vi "Virtual_Oscilloscope.vi"() -> ()   [LabVIEW 2020]
uses:
  <vilib>/Analysis/3filter.llb/Filter Passband Type.ctl
  <vilib>/Analysis/2dsp.llb/1D Convolution (DBL).vi
  <vilib>/measure/maspectr.llb/FFT Spectrum (Mag-Phase) for 1 Chan.vi
  <vilib>/Analysis/3filter.llb/Butterworth Filter (DBL).vi
  <vilib>/Analysis/3filter.llb/Chebyshev Filter (DBL).vi
  <vilib>/measure/NI_MABase.lvlib
  <vilib>/Analysis/NI_AALPro.lvlib
  <vilib>/Analysis/NI_AALBase.lvlib
  <vilib>/measure/NI_MAPro.lvlib
panel:
  in  "选项卡控件":enum32{"波形生成", "波形运算", "波形处理"}(tab)
  in  "占空比 3":dbl=50.0 caption="方波占空比(%)" format="%0.2f"
  in  "相位 3":dbl caption="相位" format="%.2p"
  in  "幅值 3":dbl=1.0 caption="幅值" format="%0.2p"
  in  "频率 3":dbl=10.0 caption="频率" format="%0.2p"
  out "CH1":waveform(dbl)(graph)
  in  "CH1波形":T1(ring)
  in  "CH1频率":i32(knob) scale=0.0..100.0
  in  "CH1幅值":i32(knob) scale=0.0..220.0
  in  "CH1相位":i32(knob) scale=0.0..180.0
  in  "CH1占空比":i32(knob) scale=0.0..100.0
  in  "采样数":dbl(slide) scale=1000.0..2000.0
  in  "采样频率":dbl(slide) scale=1000.0..2000.0
  in  "CH1-1":dbl(slide) scale=0.0..1.0
  in  "?":i32(knob) scale=1.0..7.0
  in  "Fs":dbl=1000.0 format="%.2p"
  in  "#s":dbl=1000.0 caption="采样数"
  in  "占空比 2":dbl=50.0 caption="方波占空比(%)" format="%0.2f"
  in  "相位 2":dbl caption="相位" format="%.2p"
  in  "幅值 2":dbl=1.0 caption="幅值" format="%0.2p"
  in  "频率 2":dbl=10.0 caption="频率" format="%0.2p"
  out "CH2":waveform(dbl)(graph)
  in  "CH2波形":T1(ring)
  in  "CH2-1":dbl(slide) scale=0.0..1.0
  in  "CH2幅值":i32(knob) scale=0.0..220.0
  in  "CH2相位":i32(knob) scale=0.0..180.0
  in  "CH2占空比":i32(knob) scale=0.0..100.0
  in  "CH2频率":i32(knob) scale=0.0..100.0
  in  "?":i32(knob) scale=1.0..7.0
  out "X-Y图":cluster{"Y":dbl[], "Y":dbl[]}(graph)
  in  "字符串":string
  in  "抵消":bool
  in  "叠加":bool
  in  "卷积":bool
  out "频率 5":dbl=10.0 caption="CH2频率" format="%0.2p"
  out "幅值 5":dbl=1.0 caption="CH2幅值" format="%0.2p"
  out "相位 5":dbl caption="CH2相位" format="%.2p"
  in  "处理后波形-1":dbl(slide) scale=0.0..1000.0
  in  "CH2-2":dbl(slide) scale=0.0..1.0
  out "处理后波形":dbl[](graph)
  out "CH2波形显示":waveform(dbl)(graph)
  out "CH1波形显示":waveform(dbl)(graph)
  in  "CH1-2":dbl(slide) scale=0.0..1.0
  out "频率 4":dbl=10.0 caption="CH1频率" format="%0.2p"
  out "幅值 4":dbl=1.0 caption="CH1幅值" format="%0.2p"
  out "相位 4":dbl caption="CH1相位" format="%.2p"
  out "滤波方式":enum16{"Butterworth", "Chebyshev"}(ring)
  out "滤波后FTT":cluster{"f0":dbl, "df":dbl, "magnitude":dbl[]}(graph)
  out "滤波后":dbl[](graph)
  in  "fh":dbl(slide) scale=1.0..10.0
  in  "FL":dbl(slide) scale=1.0..10.0
  in  "order":i32(knob) scale=0.0..10.0
  in  "fs":i32(knob) scale=0.0..100.0
  in  "滤波器类型":i32(knob) scale=1.0..4.0
  in  "滤波方式":i32(knob) scale=1.0..2.0
  in  "滤波后FTT":dbl(slide) scale=0.0..1.0
  out "滤波前FFT":cluster{"f0":dbl, "df":dbl, "magnitude":dbl[]}(graph)
  in  "滤波前FTT":dbl(slide) scale=0.0..1.0
  in  "滤波后":dbl(slide) scale=0.0..1000.0
  out "滤波前":dbl[](graph)
  in  "滤波前":dbl(slide) scale=0.0..1000.0
  in  "order":i32=2 caption="阶数"
  in  "filter type":T2 caption="滤波器类型"
  in  "low cutoff freq: fl":dbl=0.12500000000000006 caption="低截止频率:fl" format="%0.4f"
  in  "high cutoff freq: fh":dbl=0.45000000000000007 caption="高截止频率:fh" format="%0.2f"
  in  "sampling freq: fs":dbl=1.0 caption="采样频率:fs" format="%0.2f"
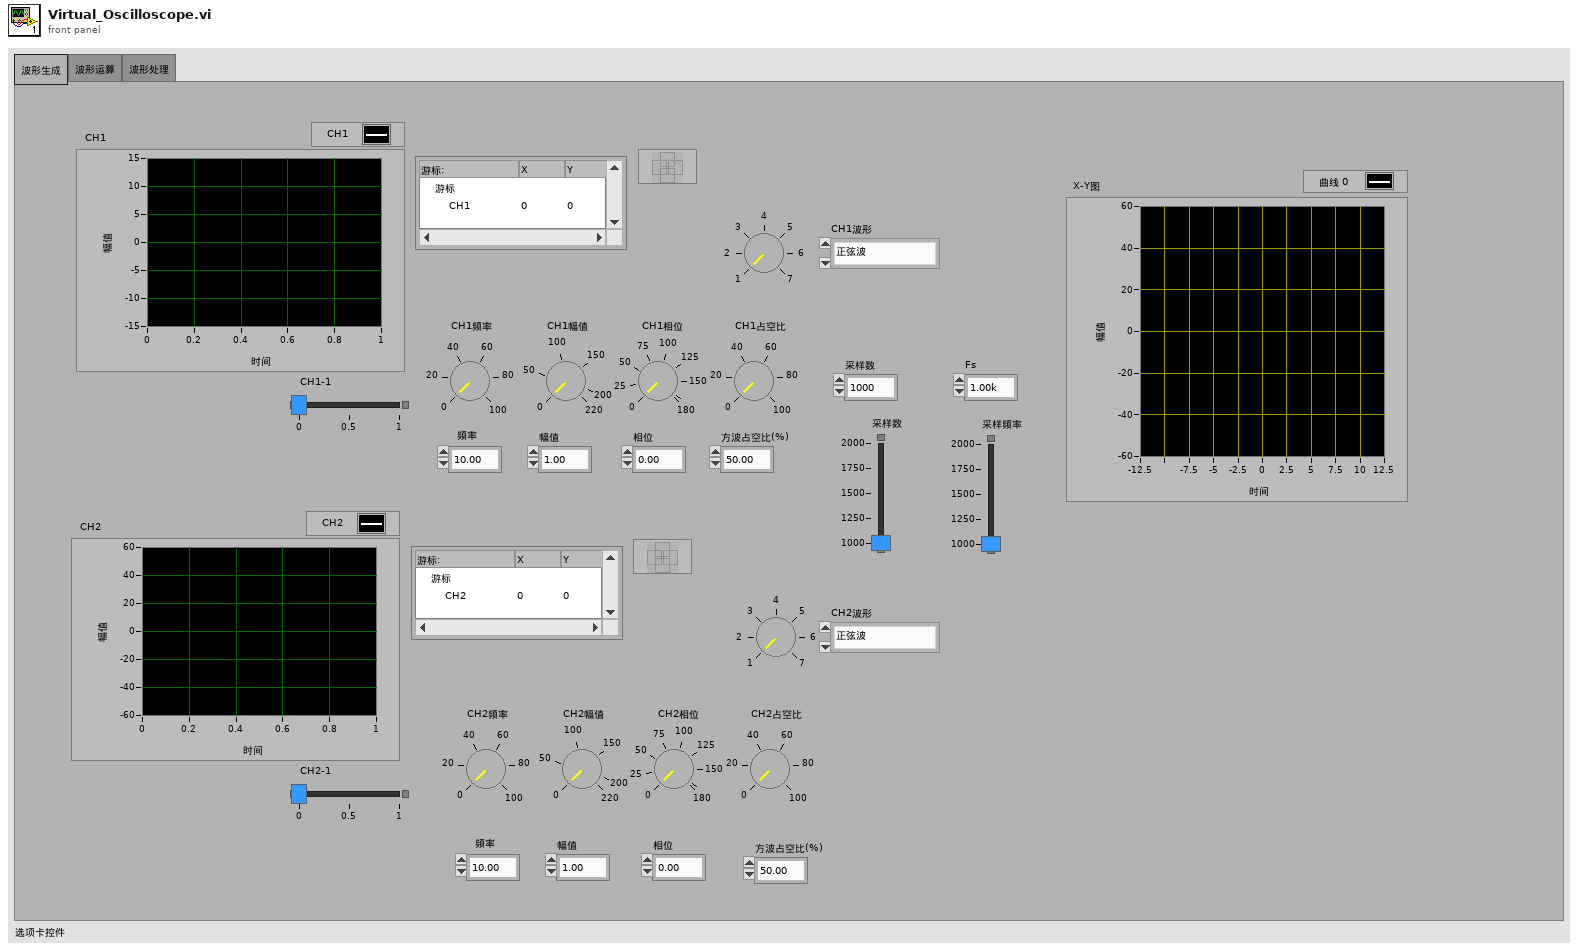
[diagram p1: front panel]
types:
  T1 = enum16{"正弦波", "三角波", "方波", "锯齿波", "高斯白噪声", "均匀白噪声", "周期噪声"}
  T2 = typedef "NI_AALBase.lvlib/Filter Passband Type.ctl" = enum32{"Lowpass", "Highpass", "Bandpass", "Bandstop"}
  T3 = enum16{"Sine Wave", "Triangle Wave", "Square Wave", "Sawtooth Wave"}
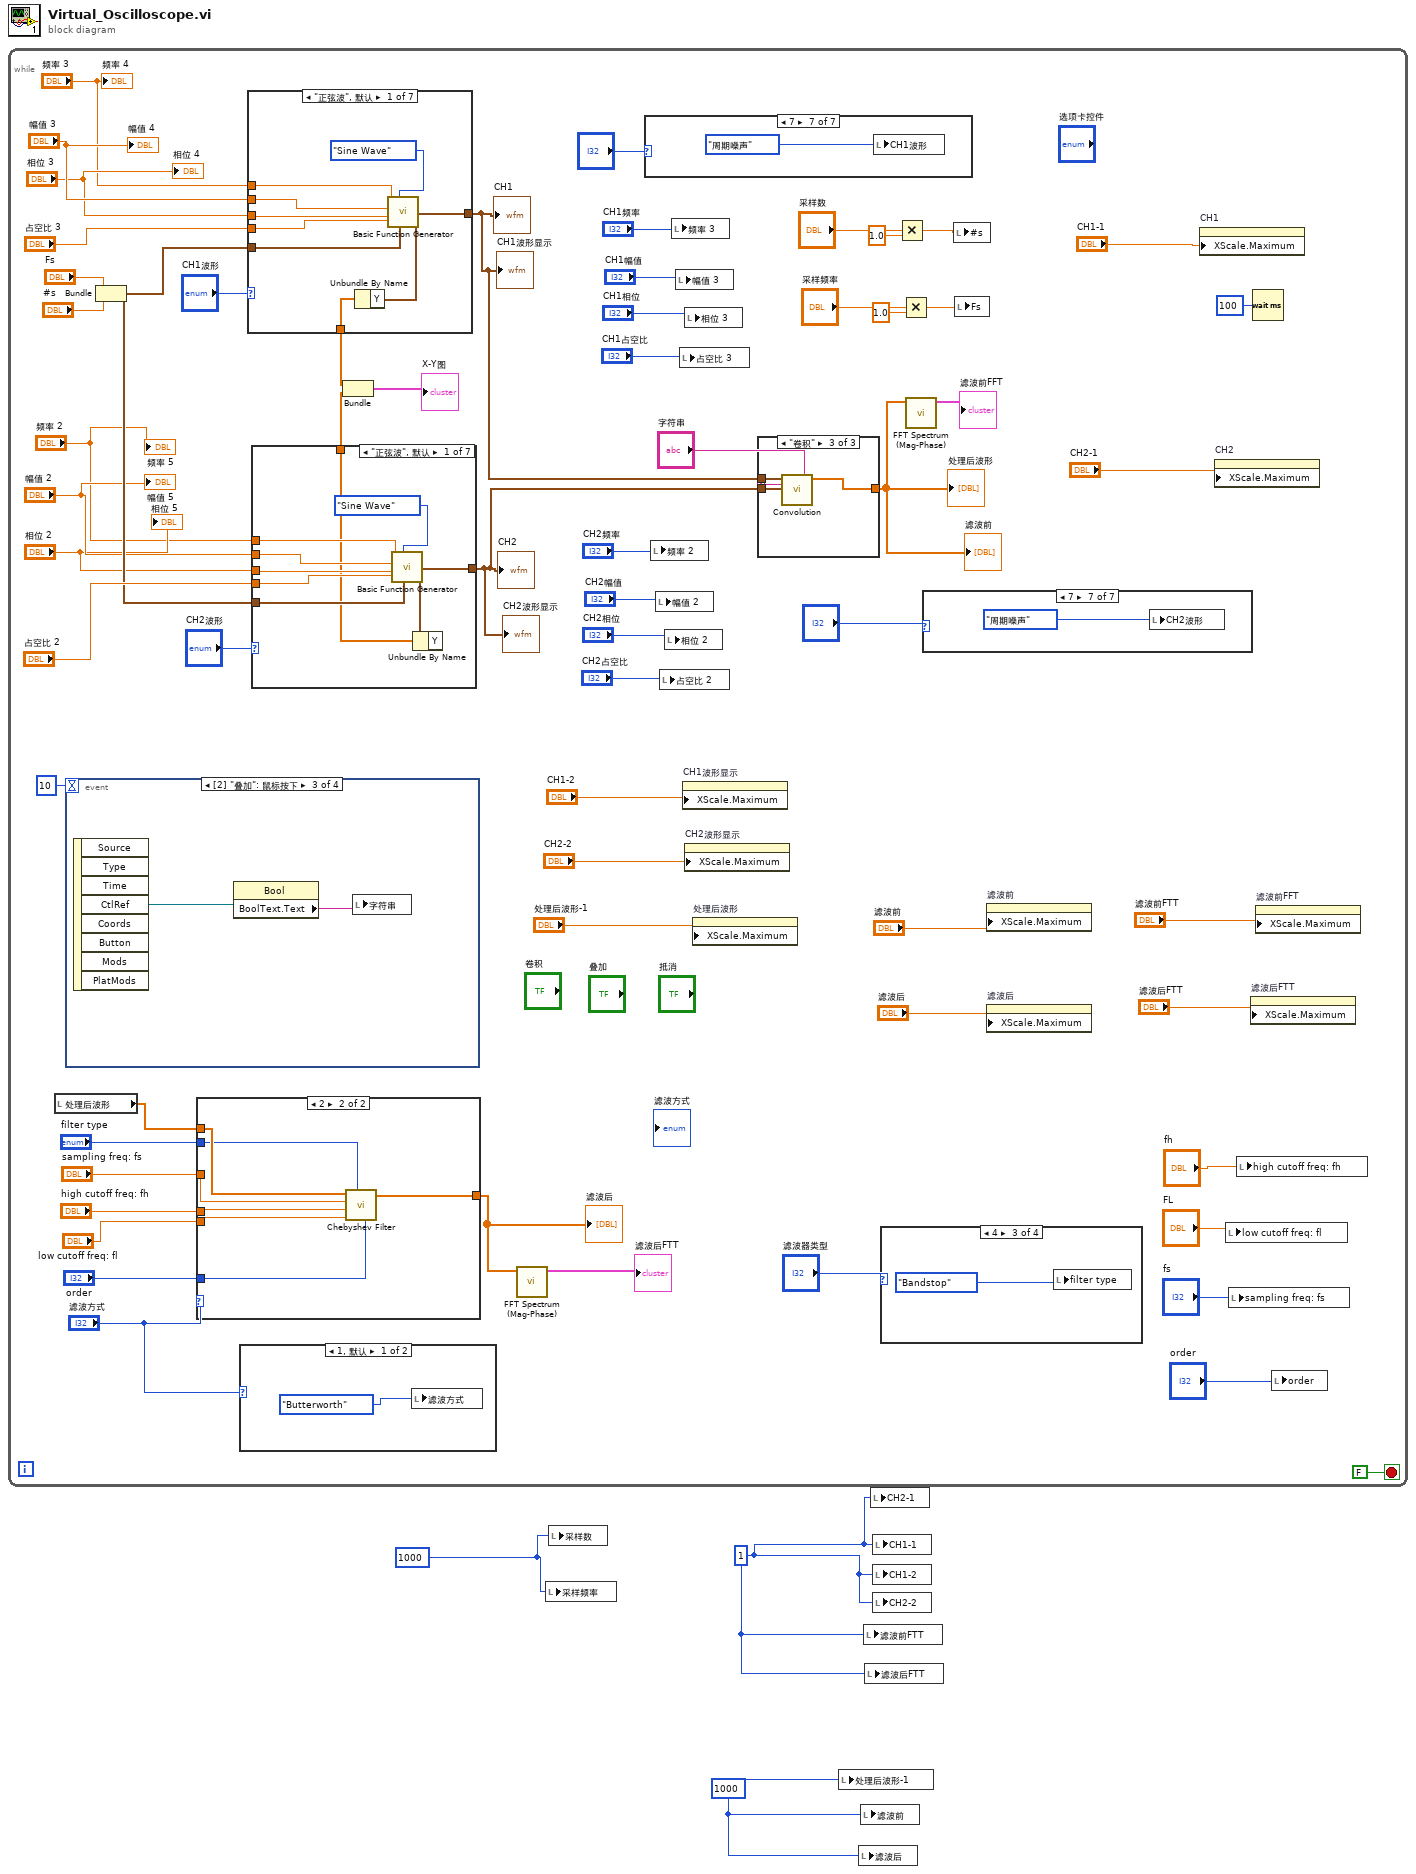
[diagram p0: block diagram]
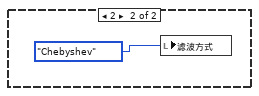
[diagram p2: hidden frame]
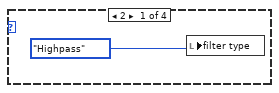
[diagram p3: hidden frame]
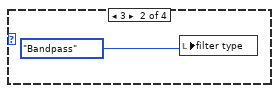
[diagram p4: hidden frame]
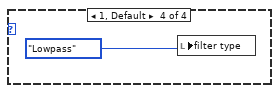
[diagram p5: hidden frame]
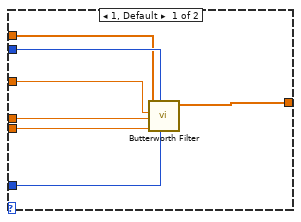
[diagram p6: hidden frame]
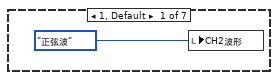
[diagram p7: hidden frame]
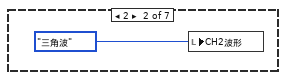
[diagram p8: hidden frame]
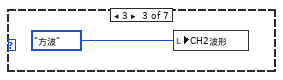
[diagram p9: hidden frame]
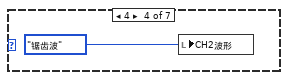
[diagram p10: hidden frame]
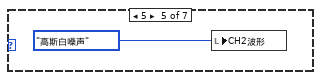
[diagram p11: hidden frame]
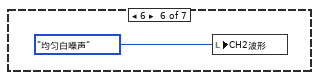
[diagram p12: hidden frame]
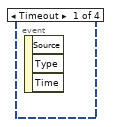
[diagram p13: hidden frame]
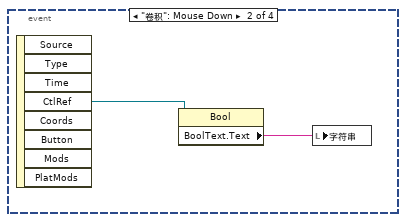
[diagram p14: hidden frame]
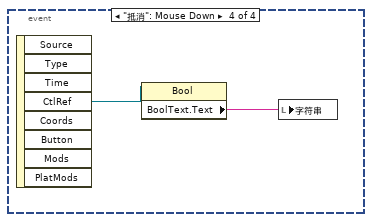
[diagram p15: hidden frame]
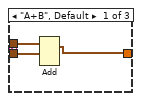
[diagram p16: hidden frame]
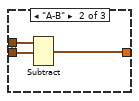
[diagram p17: hidden frame]
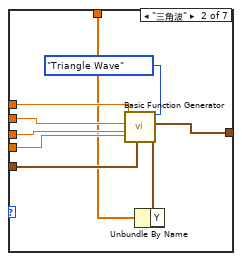
[diagram p18: hidden frame]
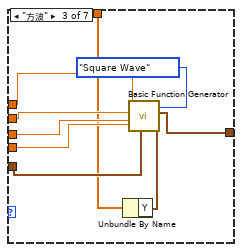
[diagram p19: hidden frame]
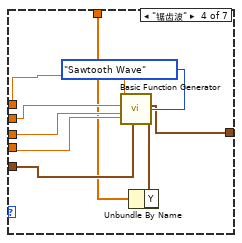
[diagram p20: hidden frame]
diagram:
  w1 = 1000
  w2 = 1
  w3 = 1000
  n1 = while {
    stop <- FALSE stop-if-true
    n2 = local read "处理后波形"() -> (w10:dbl[])
    n3 = event shown="[2] \"叠加\": 鼠标按下" {
      selector: _ -> [_ _ _ _]
      dyn-events: _ -> [_ _ _ _]
      timeout: 10 -> [_ _ _ _]
      event Timeout {
        n4 = event-data() -> ()  [unwired: 1 in, 3 out]
      }
      event "卷积": Mouse Down {
        n5 = event-data() -> ("CtlRef"=w95:refnum<vi>)  [unwired: 1 in, 7 out]
        n6 = property class="Bool"(reference=w95) -> ("BoolText.Text"=w94:string)  [unwired: 1 in, 2 out]
        n7 = local write "字符串"(w94) -> ()
      }
      event "叠加": Mouse Down {
        n8 = event-data() -> ("CtlRef"=w96:refnum<vi>)  [unwired: 1 in, 7 out]
        n9 = property class="Bool"(reference=w96) -> ("BoolText.Text"=w97:string)  [unwired: 1 in, 2 out]
        n10 = local write "字符串"(w97) -> ()
      }
      event "抵消": Mouse Down {
        n11 = event-data() -> ("CtlRef"=w98:refnum<vi>)  [unwired: 1 in, 7 out]
        n12 = property class="Bool"(reference=w98) -> ("BoolText.Text"=w99:string)  [unwired: 1 in, 2 out]
        n13 = local write "字符串"(w99) -> ()
      }
    }
    n14 = Bundle("Fs"="Fs", "#s"="#s") -> (w45:cluster{"Fs":dbl, "#s":dbl})  [unwired: 1 in]
    n15 = case shown="2" "滤波方式" {
      tunnel: "order" -> [w75 w80]
      tunnel: "filter type" -> [w79 w84]
      tunnel: "low cutoff freq: fl" -> [w78 w81]
      tunnel: "high cutoff freq: fh" -> [w77 w82]
      tunnel: "sampling freq: fs" -> [w76 w83]
      tunnel: [w74 w86] -> w8
      tunnel: w10 -> [w73 w85]
      frame 1, Default {
        n16 = call-poly <vilib>:"Butterworth Filter.vi"("order"=w75, "filter type"=w79, "low cutoff freq: fl"=w78, "high cutoff freq: fh"=w77, "sampling freq: fs"=w76, "X"=w73) -> ("Filtered X"=w74:dbl[])  [unwired: 2 in, 1 out]
      }
      frame 2 {
        n17 = call-poly <vilib>:"Chebyshev Filter.vi"("order"=w80, "filter type"=w84, "low cutoff freq: fl"=w81, "high cutoff freq: fh"=w82, "sampling freq: fs"=w83, "X"=w85) -> ("Filtered X"=w86:dbl[])  [unwired: 4 in, 1 out]
      }
    }
    "滤波后" <- w8
    n18 = case shown="1, 默认" "滤波方式" {
      frame 1, Default {
        n19 = local write "滤波方式"(enum16{"Butterworth", "Chebyshev"}."Butterworth" ("枚举 2")) -> ()
      }
      frame 2 {
        n20 = local write "滤波方式"(enum16{"Butterworth", "Chebyshev"}."Chebyshev" ("枚举 2")) -> ()
      }
    }
    n21 = case shown="\"正弦波\", 默认" "CH1波形" {
      tunnel: w45 -> [w163 w175 w178 w186 w195 w198 w202]
      tunnel: "相位 3" -> [w164 w174 w180 w188 _ _ _]
      tunnel: "幅值 3" -> [w165 w173 w181 w189 w194 w199 w203]
      tunnel: "频率 3" -> [w166 w172 w182 w190 _ _ _]
      tunnel: "占空比 3" -> [w162 w171 w179 w187 _ _ _]
      tunnel: [w161 w169 w177 w185 w193 w197 w201] -> w36
      tunnel: [w160 w168 w176 w184 w192 w196 w200] -> w27
      frame "正弦波", Default {
        n22 = call <vilib>:"Basic Function Generator.vi"("square wave duty cycle (%)"=w162, "sampling info"=w163, "signal type"=T3."Sine Wave", "phase"=w164, "amplitude"=w165, "frequency"=w166) -> ("signal out"=w161:waveform(dbl))  [unwired: 3 in, 2 out]
        n23 = Unbundle By Name(w161) -> ("Y"=w160:dbl[])
      }
      frame "三角波" {
        n24 = call <vilib>:"Basic Function Generator.vi"("square wave duty cycle (%)"=w171, "sampling info"=w175, "signal type"=T3."Triangle Wave", "phase"=w174, "amplitude"=w173, "frequency"=w172) -> ("signal out"=w169:waveform(dbl))  [unwired: 3 in, 2 out]
        n25 = Unbundle By Name(w169) -> ("Y"=w168:dbl[])
      }
      frame "方波" {
        n26 = call <vilib>:"Basic Function Generator.vi"("square wave duty cycle (%)"=w179, "sampling info"=w178, "signal type"=T3."Square Wave", "phase"=w180, "amplitude"=w181, "frequency"=w182) -> ("signal out"=w177:waveform(dbl))  [unwired: 3 in, 2 out]
        n27 = Unbundle By Name(w177) -> ("Y"=w176:dbl[])
      }
      frame "锯齿波" {
        n28 = call <vilib>:"Basic Function Generator.vi"("square wave duty cycle (%)"=w187, "sampling info"=w186, "signal type"=T3."Sawtooth Wave", "phase"=w188, "amplitude"=w189, "frequency"=w190) -> ("signal out"=w185:waveform(dbl))  [unwired: 3 in, 2 out]
        n29 = Unbundle By Name(w185) -> ("Y"=w184:dbl[])
      }
      frame "高斯白噪声" {
        n30 = call <vilib>:"Gaussian White Noise Waveform.vi"("sampling info"=w195, "standard deviation"=w194) -> ("signal out"=w193:waveform(dbl))  [unwired: 8 in, 1 out]
        n31 = Unbundle By Name(w193) -> ("Y"=w192:dbl[])
      }
      frame "均匀白噪声" {
        n32 = call <vilib>:"Uniform White Noise Waveform.vi"("sampling info"=w198, "amplitude"=w199) -> ("signal out"=w197:waveform(dbl))  [unwired: 8 in, 1 out]
        n33 = Unbundle By Name(w197) -> ("Y"=w196:dbl[])
      }
      frame "周期噪声" {
        n34 = call <vilib>:"Periodic Random Noise Waveform.vi"("sampling info"=w202, "spectral amplitude"=w203) -> ("signal out"=w201:waveform(dbl))  [unwired: 8 in, 1 out]
        n35 = Unbundle By Name(w201) -> ("Y"=w200:dbl[])
      }
    }
    "CH1" <- w36
    "CH1波形显示" <- w36
    n36 = case shown="\"正弦波\", 默认" "CH2波形" {
      tunnel: w45 -> [w111 w124 w127 w135 w144 w147 w151]
      tunnel: "相位 2" -> [w113 w123 w129 w137 _ _ _]
      tunnel: "幅值 2" -> [w114 w122 w130 w138 w143 w148 w152]
      tunnel: "频率 2" -> [w115 w121 w131 w139 _ _ _]
      tunnel: "占空比 2" -> [w112 w120 w128 w136 _ _ _]
      tunnel: [w110 w118 w126 w134 w142 w146 w150] -> w35
      tunnel: [w109 w117 w125 w133 w141 w145 w149] -> w26
      frame "正弦波", Default {
        n37 = call <vilib>:"Basic Function Generator.vi"("square wave duty cycle (%)"=w112, "sampling info"=w111, "signal type"=T3."Sine Wave", "phase"=w113, "amplitude"=w114, "frequency"=w115) -> ("signal out"=w110:waveform(dbl))  [unwired: 3 in, 2 out]
        n38 = Unbundle By Name(w110) -> ("Y"=w109:dbl[])
      }
      frame "三角波" {
        n39 = call <vilib>:"Basic Function Generator.vi"("square wave duty cycle (%)"=w120, "sampling info"=w124, "signal type"=T3."Triangle Wave", "phase"=w123, "amplitude"=w122, "frequency"=w121) -> ("signal out"=w118:waveform(dbl))  [unwired: 3 in, 2 out]
        n40 = Unbundle By Name(w118) -> ("Y"=w117:dbl[])
      }
      frame "方波" {
        n41 = call <vilib>:"Basic Function Generator.vi"("square wave duty cycle (%)"=w128, "sampling info"=w127, "signal type"=T3."Square Wave", "phase"=w129, "amplitude"=w130, "frequency"=w131) -> ("signal out"=w126:waveform(dbl))  [unwired: 3 in, 2 out]
        n42 = Unbundle By Name(w126) -> ("Y"=w125:dbl[])
      }
      frame "锯齿波" {
        n43 = call <vilib>:"Basic Function Generator.vi"("square wave duty cycle (%)"=w136, "sampling info"=w135, "signal type"=T3."Sawtooth Wave", "phase"=w137, "amplitude"=w138, "frequency"=w139) -> ("signal out"=w134:waveform(dbl))  [unwired: 3 in, 2 out]
        n44 = Unbundle By Name(w134) -> ("Y"=w133:dbl[])
      }
      frame "高斯白噪声" {
        n45 = call <vilib>:"Gaussian White Noise Waveform.vi"("sampling info"=w144, "standard deviation"=w143) -> ("signal out"=w142:waveform(dbl))  [unwired: 8 in, 1 out]
        n46 = Unbundle By Name(w142) -> ("Y"=w141:dbl[])
      }
      frame "均匀白噪声" {
        n47 = call <vilib>:"Uniform White Noise Waveform.vi"("sampling info"=w147, "amplitude"=w148) -> ("signal out"=w146:waveform(dbl))  [unwired: 8 in, 1 out]
        n48 = Unbundle By Name(w146) -> ("Y"=w145:dbl[])
      }
      frame "周期噪声" {
        n49 = call <vilib>:"Periodic Random Noise Waveform.vi"("sampling info"=w151, "spectral amplitude"=w152) -> ("signal out"=w150:waveform(dbl))  [unwired: 8 in, 1 out]
        n50 = Unbundle By Name(w150) -> ("Y"=w149:dbl[])
      }
    }
    "CH2" <- w35
    "CH2波形显示" <- w35
    n51 = Bundle("Y"=w27, "Y"=w26) -> (→"X-Y图":cluster{"Y":dbl[], "Y":dbl[]})  [unwired: 1 in]
    n52 = call-poly <vilib>:"FFT Spectrum (Mag-Phase).vi"("time signal"=w8) -> ("magnitude"=→"滤波后FTT":cluster{"f0":dbl, "df":dbl, "magnitude":dbl[]})  [unwired: 6 in, 4 out]
    n53 = case shown="7" "?" {
      frame 1, Default {
        n54 = local write "CH1波形"(T1."正弦波" ("波形 2")) -> ()
      }
      frame 2 {
        n55 = local write "CH1波形"(T1."三角波" ("波形 2")) -> ()
      }
      frame 3 {
        n56 = local write "CH1波形"(T1."方波" ("波形 2")) -> ()
      }
      frame 4 {
        n57 = local write "CH1波形"(T1."锯齿波" ("波形 2")) -> ()
      }
      frame 5 {
        n58 = local write "CH1波形"(T1."高斯白噪声" ("波形 2")) -> ()
      }
      frame 6 {
        n59 = local write "CH1波形"(T1."均匀白噪声" ("波形 2")) -> ()
      }
      frame 7 {
        n60 = local write "CH1波形"(T1."周期噪声" ("波形 2")) -> ()
      }
    }
    n61 = local write "频率 2"("CH2频率") -> ()
    n62 = local write "幅值 2"("CH2幅值") -> ()
    n63 = local write "占空比 2"("CH2占空比") -> ()
    n64 = local write "相位 2"("CH2相位") -> ()
    n65 = local write "频率 3"("CH1频率") -> ()
    n66 = local write "幅值 3"("CH1幅值") -> ()
    n67 = local write "占空比 3"("CH1占空比") -> ()
    n68 = property on="CH1波形显示" class="WFGraph (严格)"("XScale.Maximum"="CH1-2") -> ()  [unwired: 2 in, 2 out]
    n69 = local write "相位 3"("CH1相位") -> ()
    n70 = property on="CH2波形显示" class="WFGraph (严格)"("XScale.Maximum"="CH2-2") -> ()  [unwired: 2 in, 2 out]
    n71 = property on="处理后波形" class="WFGraph (严格)"("XScale.Maximum"="处理后波形-1") -> ()  [unwired: 2 in, 2 out]
    n72 = case shown="\"卷积\"" "字符串" {
      tunnel: w36 -> [w102 w105 w108]
      tunnel: w35 -> [w101 w104 w107]
      tunnel: [w100 w103 w106] -> w12
      frame "A+B", Default {
        n73 = Add(1:w101, 2:w102) -> (0:w100:waveform(dbl))  [unwired: 1 in, 1 out]
      }
      frame "A-B" {
        n74 = Subtract(1:w104, 2:w105) -> (0:w103:waveform(dbl))  [unwired: 1 in, 1 out]
      }
      frame "卷积" {
        n75 = call-poly <vilib>:"Convolution.vi"("Y"=w107, "X"=w108) -> ("X * Y"=w106:dbl[])  [unwired: 8 in, 1 out]
      }
    }
    "处理后波形" <- w12
    "滤波前" <- w12
    n76 = case shown="4" "滤波器类型" {
      frame 2 {
        n77 = local write "filter type"(Filter_Passband_Type."Highpass" ("filter type 2")) -> ()
      }
      frame 3 {
        n78 = local write "filter type"(Filter_Passband_Type."Bandpass" ("filter type 2")) -> ()
      }
      frame 4 {
        n79 = local write "filter type"(Filter_Passband_Type."Bandstop" ("filter type 2")) -> ()
      }
      frame 1, Default {
        n80 = local write "filter type"(Filter_Passband_Type."Lowpass" ("filter type 2")) -> ()
      }
    }
    n81 = Multiply(x="采样数", y=1.0) -> (x*y=w57:dbl)
    n82 = Multiply(x="采样频率", y=1.0) -> (x*y=w56:dbl)
    n83 = call-poly <vilib>:"FFT Spectrum (Mag-Phase).vi"("time signal"=w12) -> ("magnitude"=→"滤波前FFT":cluster{"f0":dbl, "df":dbl, "magnitude":dbl[]})  [unwired: 6 in, 4 out]
    n84 = case shown="7" "?" {
      frame 1, Default {
        n85 = local write "CH2波形"(T1."正弦波" ("波形 2")) -> ()
      }
      frame 2 {
        n86 = local write "CH2波形"(T1."三角波" ("波形 2")) -> ()
      }
      frame 3 {
        n87 = local write "CH2波形"(T1."方波" ("波形 2")) -> ()
      }
      frame 4 {
        n88 = local write "CH2波形"(T1."锯齿波" ("波形 2")) -> ()
      }
      frame 5 {
        n89 = local write "CH2波形"(T1."高斯白噪声" ("波形 2")) -> ()
      }
      frame 6 {
        n90 = local write "CH2波形"(T1."均匀白噪声" ("波形 2")) -> ()
      }
      frame 7 {
        n91 = local write "CH2波形"(T1."周期噪声" ("波形 2")) -> ()
      }
    }
    n92 = local write "#s"(w57) -> ()
    n93 = local write "Fs"(w56) -> ()
    n94 = property on="滤波前" class="WFGraph (严格)"("XScale.Maximum"="滤波前") -> ()  [unwired: 2 in, 2 out]
    n95 = property on="滤波后" class="WFGraph (严格)"("XScale.Maximum"="滤波后") -> ()  [unwired: 2 in, 2 out]
    n96 = property on="CH1" class="WFGraph (严格)"("XScale.Maximum"="CH1-1") -> ()  [unwired: 2 in, 2 out]
    n97 = property on="CH2" class="WFGraph (严格)"("XScale.Maximum"="CH2-1") -> ()  [unwired: 2 in, 2 out]
    n98 = local write "low cutoff freq: fl"("FL") -> ()
    n99 = local write "sampling freq: fs"("fs") -> ()
    n100 = local write "high cutoff freq: fh"("fh") -> ()
    n101 = property on="滤波后FTT" class="WFGraph (严格)"("XScale.Maximum"="滤波后FTT") -> ()  [unwired: 2 in, 2 out]
    n102 = Wait (ms)(milliseconds to wait=u32 100 ("等待时间（毫秒）")) -> ()  [unwired: 1 out]
    n103 = property on="滤波前FFT" class="WFGraph (严格)"("XScale.Maximum"="滤波前FTT") -> ()  [unwired: 2 in, 2 out]
    n104 = local write "order"("order") -> ()
    "频率 4" <- "频率 3"
    "幅值 4" <- "幅值 3"
    "相位 4" <- "相位 3"
    "相位 5" <- "相位 2"
    "幅值 5" <- "幅值 2"
    "频率 5" <- "频率 2"
  }
  n105 = local write "采样频率"(w3) -> ()
  n106 = local write "采样数"(w3) -> ()
  n107 = local write "处理后波形-1"(w1) -> ()
  n108 = local write "滤波后"(w1) -> ()
  n109 = local write "滤波前"(w1) -> ()
  n110 = local write "滤波前FTT"(w2) -> ()
  n111 = local write "滤波后FTT"(w2) -> ()
  n112 = local write "CH2-1"(w2) -> ()
  n113 = local write "CH1-1"(w2) -> ()
  n114 = local write "CH1-2"(w2) -> ()
  n115 = local write "CH2-2"(w2) -> ()
